vi "test protocol version fallback.vi"(8 "error in (no error)":errorcluster) -> (0 "error out":errorcluster, 3 "body":string)   [LabVIEW 2020, in "MCP Server tests.lvlib"]
doc: "If the client asks for a protocol version the server does not support, initialize answers with the first entry of Supported Protocol Versions.vi, the newest version the server supports."
uses:
  MCP Server tests.lvlib
  d0ab81eb-4137-4fbe-b0df-76d3e507edfb.vi
  <vilib>/JDP Science/JSONtext/Next JSON Value.vi
  <vilib>/JDP Science/JSONtext/String Subset.vi
  <vilib>/JDP Science/JSONtext/Parsing/Advance past next JSON Value (inlined COPY).vi
  <vilib>/JDP Science/JSONtext/Parsing/Advance past whitespace.vi
  <vilib>/JDP Science/JSONtext/Parsing/Advance past String.vi
  <vilib>/JDP Science/JSONtext/Parsing/Advance past Number.vi
  <vilib>/JDP Science/JSONtext/Parsing/Advance past Line Ending.vi
  <vilib>/JDP Science/JSONtext/Parsing/Parse Full Path or Item Name.vi
  <vilib>/JDP Science/JSONtext/Parsing/Advance past Array.vi
  <vilib>/JDP Science/JSONtext/Parsing/Advance past Object.vi
  <vilib>/JDP Science/JSONtext/support/Error Cluster From Code.vi
  <vilib>/JDP Science/JSONtext/Offset/Find Item Locations by Path.vi
  <vilib>/JDP Science/JSONtext/JSON text to Variant.vi
  <vilib>/JDP Science/JSONtext/LVClass Serializer/JSONtext LVClass Serializer.lvclass
  <vilib>/addons/_JKI Toolkits/Caraya/classes/Test/Test.lvclass
  <vilib>/JDP Science/JSONtext/JSONtext.lvlib
  <vilib>/addons/_JKI Toolkits/Caraya/classes/Assert/Assert.lvclass
  src/MCP Server/MCP Server.lvlib
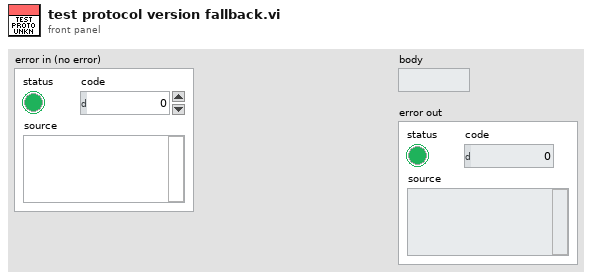
[diagram p1: front panel]
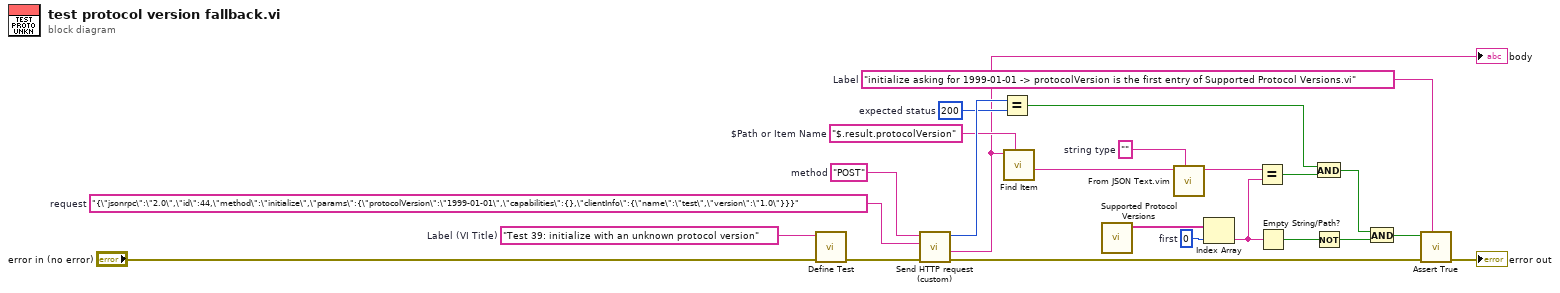
[diagram p0: block diagram]
diagram:
  w3 = "initialize asking for 1999-01-01 -> protocolVersion is the first entry of Supported Protocol Versions.vi"  # Label
  w13 = ""  # string type
  w15 = 0  # first
  w17 = "$.result.protocolVersion"  # $Path or Item Name
  w18 = 200  # expected status
  w21 = "{\"jsonrpc\":\"2.0\",\"id\":44,\"method\":\"initialize\",\"params\":{\"protocolVersion\":\"1999-01-01\",\"capabilities\":{},\"clientInfo\":{\"name\":\"test\",\"version\":\"1.0\"}}}"  # request
  w22 = "POST"  # method
  w24 = "Test 39: initialize with an unknown protocol version"  # Label (VI Title)
  n1 = call <vilib>:"Define Test.vi"("error in (no error)"="error in (no error)", "Label (VI Title)"=w24) -> ("error out"=w20:errorcluster)  [unwired: 8 in, 1 out]
  n2 = call "Send HTTP request (custom).vi"("error in (no error)"=w20, "request"=w21, "method"=w22) -> ("error out"=w4:errorcluster, "response"=w2:string, "status code"=w19:i32)  [unwired: 5 in, 1 out]
  "body" <- w2
  n3 = Equal?(x=w19, y=w18) -> (x = y?=w9:bool)
  n4 = call <vilib>:"Find Item.vi"("$Path or Item Name"=w17, "JSON"=w2) -> ("<JSON>"=w14:string)  [unwired: 6 in, 3 out]
  n5 = call "Supported Protocol Versions.vi"() -> ("supported versions"=w16:string[])  [unwired: 11 in]
  n6 = call "From JSON Text.vim"("Data Type and Default Value"=w13, "JSON"=w14) -> ("Data out"=w12:string)  [unwired: 8 in, 1 out]
  n7 = Index Array(array=w16, index=w15) -> (element=w11:string)
  n8 = Equal?(x=w12, y=w11) -> (x = y?=w8:bool)
  n9 = Empty String/Path?(string/path=w11) -> (empty?=w10:bool)
  n10 = And(x=w9, y=w8) -> (x .and. y?=w7:bool)
  n11 = Not(x=w10) -> (.not. x?=w6:bool)
  n12 = And(x=w7, y=w6) -> (x .and. y?=w5:bool)
  n13 = call <vilib>:"Assert True.vi"("Label"=w3, "error in (no error)"=w4, "True?"=w5) -> ("error out"=→"error out":errorcluster)  [unwired: 7 in, 1 out]
